vi "Moviment depredadors.vi"(6 "Numeric":dbl, 9 "Numeric 2":dbl, 10 "Array":dbl[](array[numeric]), 11 "Array 2":dbl[](array[numeric])) -> (1 "Array 4":bool[](array[boolean]), 2 "Array 3":dbl[](array[numeric]), 3 "Array 5":dbl[](array[numeric]))   [LabVIEW 2023]
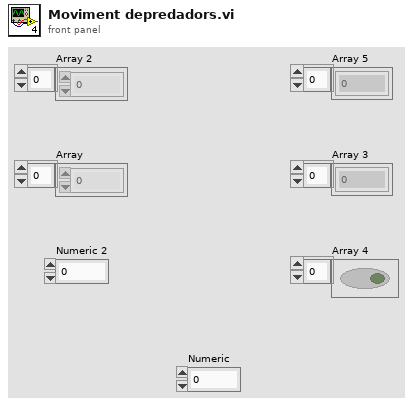
[diagram p1: front panel]
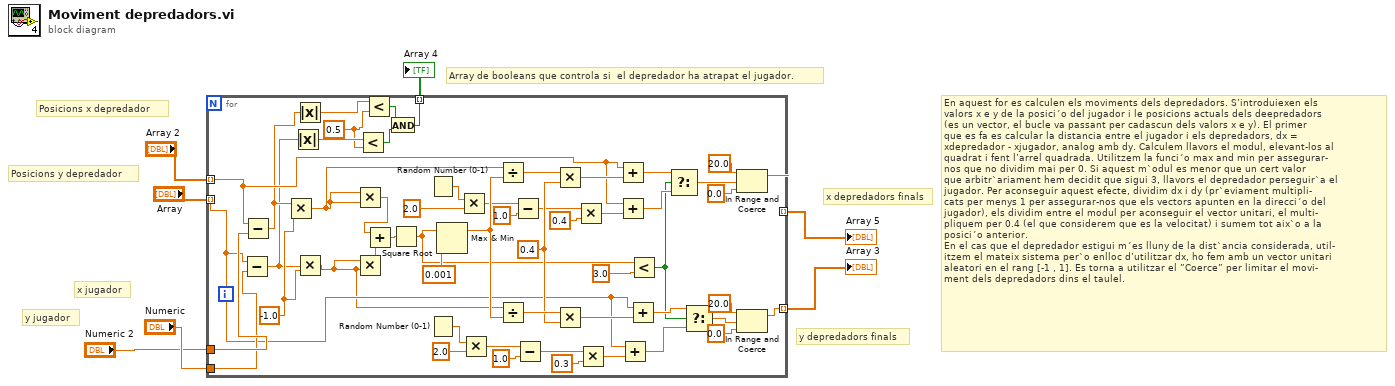
[diagram p0: block diagram]
diagram:
  # "En aquest for es calculen els moviments dels depredadors. S’introduiexen els\nvalors x e y de la posici´o del jugador i le posicions actuals dels deepredadors\n(es un vector, el bucle va passant per cadascun dels valors x e y). El primer\nque es fa es calcular la distancia entre el jugador i els depredadors, dx =\nxdepredador - xjugador, analog amb dy. Calculem llavors el modul, elevant-los al\nquadrat i fent l’arrel quadrada. Utilitzem la funci´o max and min per assegurar-\nnos que no dividim mai per 0. Si aquest m`odul es menor que un cert valor\nque arbitr`ariament hem decidit que sigui 3, llavors el depredador perseguir`a el\njugador. Per aconseguir aquest efecte, dividim dx i dy (pr`eviament multipli-\ncats per menys 1 per assegurar-nos que els vectors apunten en la direcci´o del\njugador), els dividim entre el modul per aconseguir el vector unitari, el multi-\npliquem per 0.4 (el que considerem que es la velocitat) i sumem tot aix`o a la\nposici´o anterior.\nEn el cas que el depredador estigui m´es lluny de la dist`ancia considerada, util-\nitzem el mateix sistema per`o enlloc d’utilitzar dx, ho fem amb un vector unitari\naleatori en el rang [-1 , 1]. Es torna a utilitzar el ”Coerce” per limitar el movi-\nment dels depredadors dins el taulel."
  # "y depredadors finals"
  # "x depredadors finals"
  # "Array de booleans que controla si  el depredador ha atrapat el jugador."
  # "y jugador"
  # "x jugador"
  # "Posicions y depredador"
  # "Posicions x depredador"
  n1 = for {
    tunnel: "Numeric 2" -> [w24]
    tunnel: "Numeric" -> [w23]
    tunnel: "Array" -> [w18] mode=indexing
    tunnel: "Array 2" -> [w19] mode=indexing
    tunnel: [w22] -> w1 mode=indexing
    tunnel: [w21] -> w3 mode=indexing
    tunnel: [w8] -> w2 mode=indexing
    w11 = 0.5
    w20 = -1.0
    w54 = 0.4
    n2 = Subtract(x=w18, y=w23) -> (x-y=w14:dbl)
    n3 = Subtract(x=w19, y=w24) -> (x-y=w15:dbl)
    n4 = Multiply(x=w15, y=w20) -> (x*y=w17:dbl)
    n5 = Absolute Value(x=w14) -> (abs(x)=w12:dbl)
    n6 = Absolute Value(x=w15) -> (abs(x)=w13:dbl)
    n7 = Multiply(x=w14, y=w20) -> (x*y=w16:dbl)
    n8 = Multiply(x=w17, y=w17) -> (x*y=w61:dbl)
    n9 = Multiply(x=w16, y=w16) -> (x*y=w60:dbl)
    n10 = Less?(x=w12, y=w11) -> (x < y?=w9:bool)
    n11 = Less?(x=w13, y=w11) -> (x < y?=w10:bool)
    n12 = Add(x=w61, y=w60) -> (x+y=w59:dbl)
    n13 = And(x=w10, y=w9) -> (x .and. y?=w8:bool)
    n14 = Square Root(x=w59) -> (sqrt(x)=w25:dbl)
    n15 = Random Number (0-1)() -> (number: 0 to 1=w43:dbl)
    n16 = Random Number (0-1)() -> (number: 0 to 1=w50:dbl)
    n17 = Max & Min(x=w25, y=0.001) -> (max(x,y)=w56:dbl)  [unwired: 1 out]
    n18 = Multiply(x=w43, y=2.0) -> (x*y=w41:dbl)
    n19 = Multiply(x=w50, y=2.0) -> (x*y=w48:dbl)
    n20 = Divide(x=w17, y=w56) -> (x/y=w53:dbl)
    n21 = Divide(x=w16, y=w56) -> (x/y=w55:dbl)
    n22 = Subtract(x=w41, y=1.0) -> (x-y=w39:dbl)
    n23 = Subtract(x=w48, y=1.0) -> (x-y=w46:dbl)
    n24 = Multiply(x=w53, y=w54) -> (x*y=w52:dbl)
    n25 = Multiply(x=w55, y=w54) -> (x*y=w51:dbl)
    n26 = Multiply(x=w39, y=0.4) -> (x*y=w37:dbl)
    n27 = Multiply(x=w46, y=0.3) -> (x*y=w44:dbl)
    n28 = Add(x=w19, y=w52) -> (x+y=w33:dbl)
    n29 = Add(x=w19, y=w37) -> (x+y=w34:dbl)
    n30 = Add(x=w18, y=w44) -> (x+y=w36:dbl)
    n31 = Add(x=w18, y=w51) -> (x+y=w35:dbl)
    n32 = Less?(x=w25, y=3.0) -> (x < y?=w32:bool)
    n33 = Select(t=w33, s=w32, f=w34) -> (s? t:f=w30:dbl)
    n34 = Select(t=w35, s=w32, f=w36) -> (s? t:f=w31:dbl)
    n35 = In Range and Coerce(upper limit=20.0, x=w30, lower limit=0.0) -> (coerced(x)=w22:dbl)  [unwired: 1 out]
    n36 = In Range and Coerce(upper limit=20.0, x=w31, lower limit=0.0) -> (coerced(x)=w21:dbl)  [unwired: 1 out]
  }
  "Array 3" <- w3
  "Array 4" <- w2
  "Array 5" <- w1
